vi "FuncVI_Sub - vhShow - Master.vi"() -> ()   [LabVIEW 2021]
doc: "::: CalcExpress Toolkit :::\nCopyright (c) 2000-2026 Konstantin Shifershteyn. All rights reserved."
uses:
  cetypes.llb/VarMan Variable Context Handle.ctl
  <vilib>/Utility/miscctls.llb/LVBoundsTypeDef.ctl
panel:
  out "History":bool
  in  "Reversed":bool=TRUE
  out "Variable":string
  out "h_any":T1(array[cluster]) {"timestamp" format="%<%H:%M:%S%2u\n%d/%m/%Y>T"}
  out "h_a2str":T2(array[cluster]) {"timestamp" format="%<%H:%M:%S%2u\n%d/%m/%Y>T"}
  out "h_a1str":T3(array[cluster]) {"timestamp" format="%<%H:%M:%S%2u\n%d/%m/%Y>T"}
  out "h_a2cdb":T4(array[cluster]) {"value"."data" format="%.2f"; "timestamp" format="%<%H:%M:%S%2u\n%d/%m/%Y>T"}
  out "h_a1cdb":T5(array[cluster]) {"value"."data" format="%.2f"; "timestamp" format="%<%H:%M:%S%2u\n%d/%m/%Y>T"}
  out "h_cdb":T6(array[cluster]) {"value" format="%.2f"; "timestamp" format="%<%H:%M:%S%2u\n%d/%m/%Y>T"}
  out "h_a2dbl":T7(array[cluster]) {"value"."data" format="%.2f"; "timestamp" format="%<%H:%M:%S%2u\n%d/%m/%Y>T"}
  out "h_a1dbl":T8(array[cluster]) {"value"."data" format="%.2f"; "timestamp" format="%<%H:%M:%S%2u\n%d/%m/%Y>T"}
  out "h_dbl":T9(array[cluster]) caption="Variable History" {"value" format="%.2f"; "timestamp" format="%<%H:%M:%S%2u\n%d/%m/%Y>T"}
  out "h_str":T1(array[cluster]) caption="Variable History" {"timestamp" format="%<%H:%M:%S%2u\n%d/%m/%Y>T"}
  in  "name":string
  in  "vch":T10=-1
  in  "update":bool
  in  "Display style":u32(ring) items=["Normal", "'\\' Code", "Password", "Hex dump"]
  in  "Precision":u8=2
  in  "Format":u8(ring) items=["Floating point", "Scientific", "Engineering", "Binary", "Octal", "Hexadecimal", "Relative time", "Absolute time"]
  out "Var Type":i32(ring)=1 items=["String", "DBL Number", "identifier", "1D Array of DBL", "2D Array of DBL", "CDB Number", "1D Array of CDB", "2D Array of CDB", "1D Array of String", "2D Array of String", "Unknown data type"]
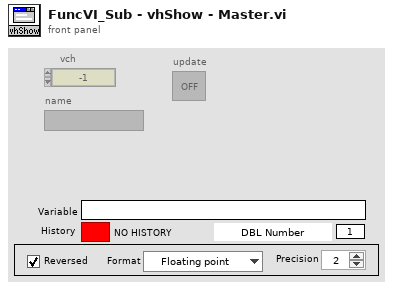
[diagram p1: front panel]
types:
  T1 = cluster{"timestamp":dbl, "value":string, "writerID":u32}[]
  T2 = cluster{"timestamp":dbl, "value":cluster{"data":string[][]}, "writerID":u32}[]
  T3 = cluster{"timestamp":dbl, "value":cluster{"data":string[]}, "writerID":u32}[]
  T4 = cluster{"timestamp":dbl, "value":cluster{"data":cdb[][]}, "writerID":u32}[]
  T5 = cluster{"timestamp":dbl, "value":cluster{"data":cdb[]}, "writerID":u32}[]
  T6 = cluster{"timestamp":dbl, "value":cdb, "writerID":u32}[]
  T7 = cluster{"timestamp":dbl, "value":cluster{"data":dbl[][]}, "writerID":u32}[]
  T8 = cluster{"timestamp":dbl, "value":cluster{"data":dbl[]}, "writerID":u32}[]
  T9 = cluster{"timestamp":dbl, "value":dbl, "writerID":u32}[]
  T10 = typedef "VarMan Variable Context Handle.ctl" = i32
  T11 = typedef "LVBoundsTypeDef.ctl" = cluster{"Width":u32, "Height":u32}
  T12 = typedef "LVPositionTypeDef.ctl" = cluster{"Left":i32, "Top":i32}
  T13 = typedef "eventvkey.ctl" = enum16{"ASCII", "Enter", "Return", "Shift", "Ctrl", "Alt", "Cmd", "Opt", "Caps", "NumLock", "Clear", "Break", "Up", "Down", "Left", "Right", "Insert", "Delete", "Home", "End", "PageUp", "PageDown", "Escape", "Help", "Pause", "ScrollLock", "F1", "F2", "F3", "F4", "F5", "F6", "F7", "F8", "F9", "F10", "F11", "F12", "F13", "F14", "F15", "F16", "F17", "F18", "F19", "F20", "F21", "F22", "F23", "F24", "Play", "VolumeUp", "VolumeDown", "Mute", "Two Byte Char"}
  T14 = cluster{"Shift":bool, "Ctrl":bool, "Alt":bool, "Cmd":bool, "Opt":bool}
  T15 = cluster{"timestamp":dbl, "value":string, "value":u32}[]
  T16 = cluster{"timestamp":dbl, "value":dbl, "value":u32}[]
  T17 = cluster{"timestamp":dbl, "value":cluster{"data":dbl[]}, "value":u32}[]
  T18 = cluster{"timestamp":dbl, "value":cluster{"data":dbl[][]}, "value":u32}[]
  T19 = cluster{"timestamp":dbl, "value":cdb, "value":u32}[]
  T20 = cluster{"timestamp":dbl, "value":cluster{"data":cdb[]}, "value":u32}[]
  T21 = cluster{"timestamp":dbl, "value":cluster{"data":cdb[][]}, "value":u32}[]
  T22 = cluster{"timestamp":dbl, "value":cluster{"data":string[]}, "value":u32}[]
  T23 = cluster{"timestamp":dbl, "value":cluster{"data":string[][]}, "value":u32}[]
  T24 = typedef "LVRectTypeDef.ctl" = cluster{"Left":i16, "Top":i16, "Right":i16, "Bottom":i16}
  T25 = cluster{"Left":i32, "Top":i32, "Right":i32, "Bottom":i32}
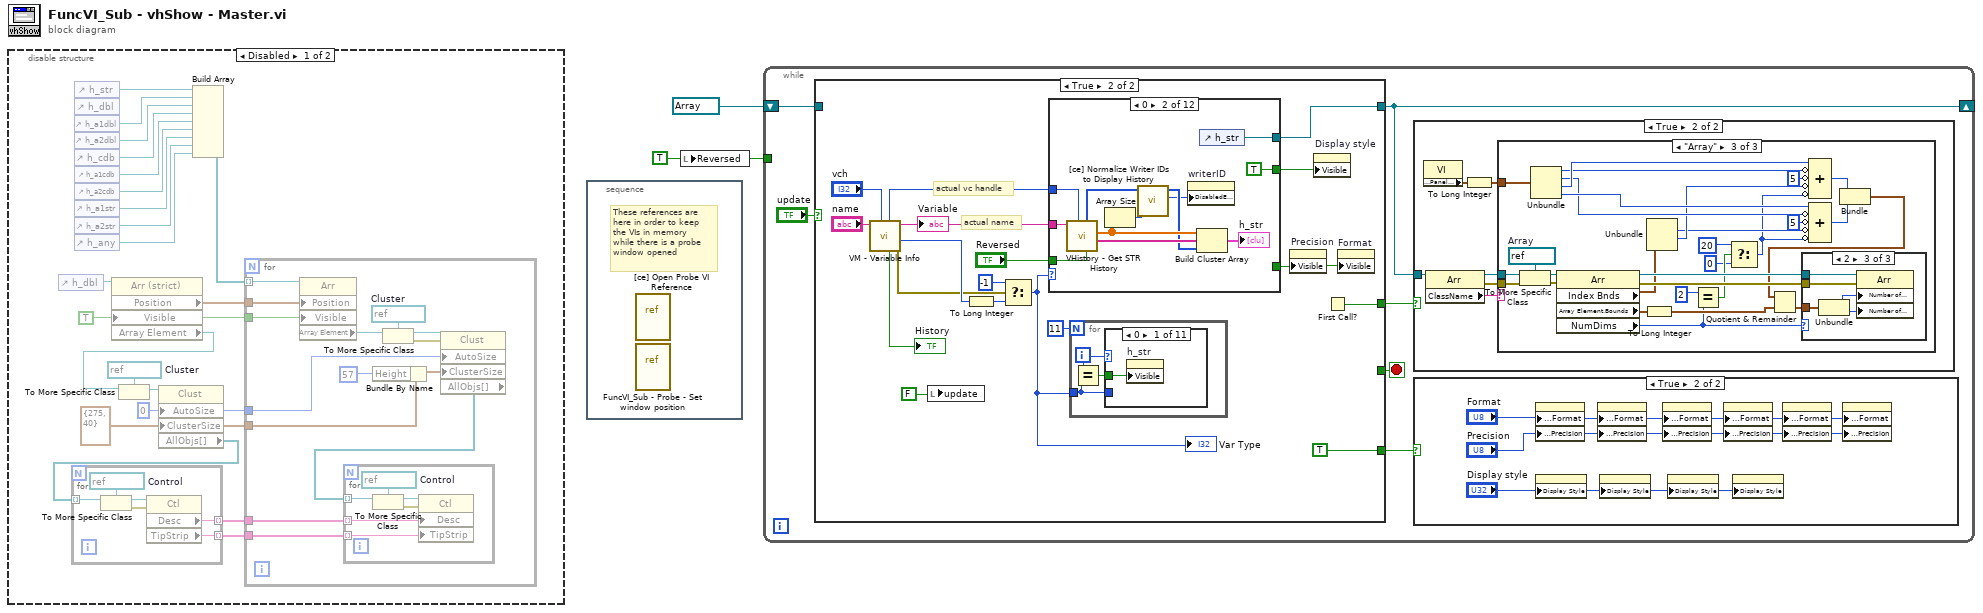
[diagram p0: block diagram]
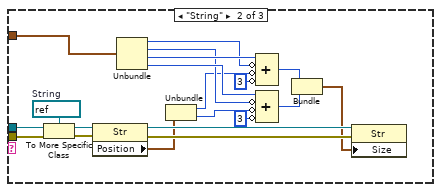
[diagram p5: hidden frame]
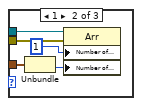
[diagram p7: hidden frame]
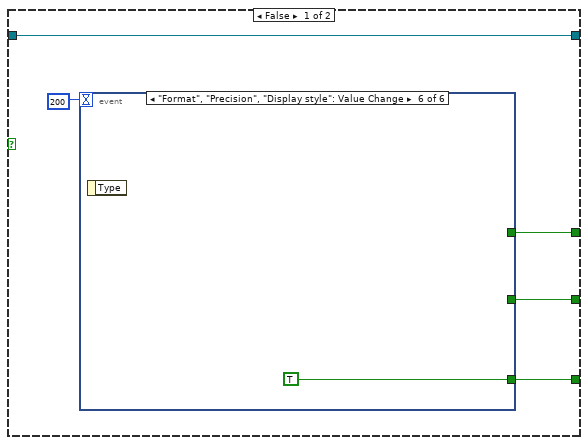
[diagram p9: hidden frame]
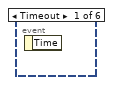
[diagram p10: hidden frame]
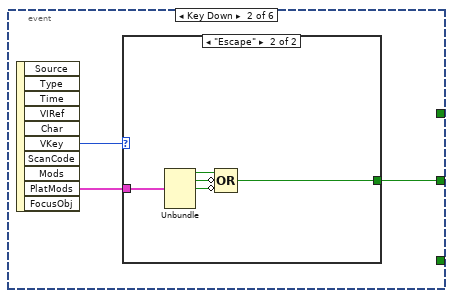
[diagram p11: hidden frame]
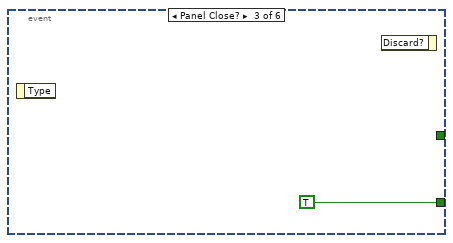
[diagram p13: hidden frame]
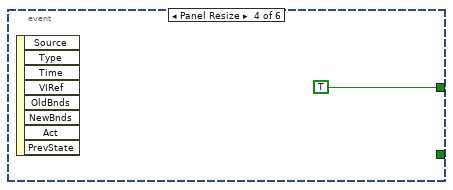
[diagram p14: hidden frame]
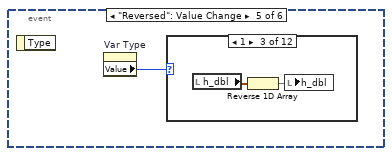
[diagram p15: hidden frame]
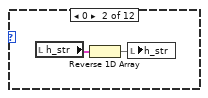
[diagram p17: hidden frame]
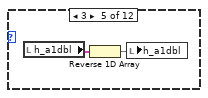
[diagram p19: hidden frame]
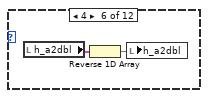
[diagram p20: hidden frame]
diagram:
  w2 = TRUE ("reversed")
  n1 = disable-structure shown="Disabled" {
    frame Disabled {
      w3 = TRUE ("Visible")
      w7 = T11 {"Width"=275, "Height"=40} ("Cluster Size")
      w8 = u32 0 ("Auto Sizing")
      w11 = refnum<vi> refnum  # Cluster
      n2 = control-ref of="h_dbl"() -> (w14:refnum<vi>)
      n3 = control-ref of="h_str"() -> (w23:refnum<vi>)
      n4 = control-ref of="h_dbl"() -> ()  [unwired: 1 out]
      n5 = control-ref of="h_a1dbl"() -> (w22:refnum<vi>)
      n6 = control-ref of="h_a2dbl"() -> (w21:refnum<vi>)
      n7 = control-ref of="h_cdb"() -> (w20:refnum<vi>)
      n8 = control-ref of="h_a1cdb"() -> (w19:refnum<vi>)
      n9 = control-ref of="h_a2cdb"() -> (w18:refnum<vi>)
      n10 = control-ref of="h_a1str"() -> (w17:refnum<vi>)
      n11 = control-ref of="h_a2str"() -> (w16:refnum<vi>)
      n12 = control-ref of="h_any"() -> (w15:refnum<vi>)
      n13 = property class="Arr (strict)"(reference=w14, "Visible"=w3) -> ("Position"=w13:T12, "Array Element"=w10:refnum<vi>)  [unwired: 1 in, 2 out]
      n14 = To More Specific Class(target class=w11, reference=w10) -> (specific class reference=w9:refnum<vi>)  [unwired: 1 in, 1 out]
      n15 = property class="Clust"(reference=w9, "AutoSize"=w8, "ClusterSize"=w7) -> ("AllObjs[]"=w6:refnum<vi>[])  [unwired: 1 in, 2 out]
      n16 = for {
        tunnel: w6 -> [w28] mode=indexing
        tunnel: [w25] -> w5 mode=indexing
        tunnel: [w24] -> w4 mode=indexing
        w29 = refnum<vi> refnum  # Control
        n17 = To More Specific Class(target class=w29, reference=w28) -> (specific class reference=w27:refnum<vi>, error out=w26:errorcluster)  [unwired: 1 in]
        n18 = property class="Ctl"(reference=w27, error in=w26) -> ("Desc"=w25:string, "TipStrip"=w24:string)  [unwired: 2 out]
      }
      n19 = Build Array(w23, w22, w21, w20, w19, w18, w17, w16, w15) -> (w12:refnum<vi>[])
      n20 = for {
        tunnel: w13 -> [w43]
        tunnel: w12 -> [w42] mode=indexing
        tunnel: w8 -> [w37]
        tunnel: w7 -> [w36]
        tunnel: w5 -> [w32]
        tunnel: w4 -> [w31]
        tunnel: w3 -> [w30]
        w41 = refnum<vi> refnum  # Cluster
        n21 = property class="Arr"(reference=w42, "Position"=w43, "Visible"=w30) -> ("Array Element"=w40:refnum<vi>)  [unwired: 1 in, 2 out]
        n22 = Bundle By Name(cluster=w36, "Height"=u32 57) -> (w35:T11)
        n23 = To More Specific Class(target class=w41, reference=w40) -> (specific class reference=w39:refnum<vi>, error out=w38:errorcluster)  [unwired: 1 in]
        n24 = property class="Clust"(reference=w39, error in=w38, "AutoSize"=w37, "ClusterSize"=w35) -> ("AllObjs[]"=w33:refnum<vi>[])  [unwired: 2 out]
        n25 = for {
          tunnel: w33 -> [w48] mode=indexing
          tunnel: w32 -> [w45] mode=indexing
          tunnel: w31 -> [w44] mode=indexing
          w49 = refnum<vi> refnum  # Control
          n26 = To More Specific Class(target class=w49, reference=w48) -> (specific class reference=w47:refnum<vi>, error out=w46:errorcluster)  [unwired: 1 in]
          n27 = property class="Ctl"(reference=w47, error in=w46, "Desc"=w45, "TipStrip"=w44) -> ()  [unwired: 2 out]
        }
      }
    }
    frame Enabled {
    }
  }
  n28 = stacked-sequence {
    frame #0 {
      # "These references are\nhere in order to keep\nthe VIs in memory\nwhile there is a probe\nwindow opened"
      n29 = vi-ref "[ce] Open Probe VI Reference.vi"() -> ()  [unwired: 1 out]
      n30 = vi-ref "FuncVI_Sub - Probe - Set window position.vi"() -> ()  [unwired: 1 out]
    }
  }
  n31 = local write "Reversed"(w2) -> ()
  n32 = while {
    tunnel: w2 -> [_]
    shift-right: [w51] -> _
    shift-left: refnum<vi> refnum ("h_str") -> [w53]
    stop <- w54 stop-if-true
    n33 = case shown="True" "update" {
      tunnel: [w127 _] -> w54
      tunnel: [w126 w162] -> w51
      tunnel: w53 -> [w126 _]
      tunnel: [w125 TRUE] -> w52
      tunnel: [w124 w161] -> w50
      frame False {
        n34 = event shown="[5] \"Format\", \"Precision\", \"Display style\": Value Change" {
          selector: _ -> [_ _ _ _ _ _]
          dyn-events: _ -> [_ _ _ _ _ _]
          timeout: 200 ("millisecond multiple") -> [_ _ _ _ _ _]
          tunnel: [_ w129 TRUE _ _ _] -> w127
          tunnel: [_ _ _ _ _ TRUE] -> w125
          tunnel: [_ _ _ TRUE _ _] -> w124
          event Timeout {
            n35 = event-data() -> ()  [unwired: 1 in, 1 out]
          }
          event Key Down {
            n36 = event-data() -> ("VKey"=w131:T13, "PlatMods"=w130:T14)  [unwired: 1 in, 8 out]
            n37 = case shown="\"Escape\"" w131 {
              tunnel: w130 -> [_ w136]
              tunnel: [_ w132] -> w129
              frame Default {
              }
              frame "Escape" {
                n38 = Unbundle(w136) -> ("Shift"=w135:bool, "Ctrl"=w134:bool, "Alt"=w133:bool)  [unwired: 2 out]
                n39 = Compound Arithmetic op=OR(w135, invert w134, invert w133) -> (w132:bool)
              }
            }
          }
          event Panel Close? {
            n40 = event-data() -> ()  [unwired: 1 in, 1 out]
            n41 = event-data() -> ()  [unwired: 2 in, 1 out]
          }
          event Panel Resize {
            n42 = event-data() -> ()  [unwired: 1 in, 8 out]
          }
          event "Reversed": Value Change {
            n43 = event-data() -> ()  [unwired: 1 in, 1 out]
            n44 = property on="Var Type" class="Ring (strict)"() -> ("Value"=w139:i32)  [unwired: 2 in, 2 out]
            n45 = case shown="1" w139 {
              frame -1 {
              }
              frame 0 {
                n46 = local read "h_str"() -> (w141:T1)
                n47 = Reverse 1D Array(array=w141) -> (reversed array=w140:T1)
                n48 = local write "h_str"(w140) -> ()
              }
              frame 1 {
                n49 = local read "h_dbl"() -> (w143:T9)
                n50 = Reverse 1D Array(array=w143) -> (reversed array=w142:T9)
                n51 = local write "h_dbl"(w142) -> ()
              }
              frame 2 {
              }
              frame 3 {
                n52 = local read "h_a1dbl"() -> (w145:T8)
                n53 = Reverse 1D Array(array=w145) -> (reversed array=w144:T8)
                n54 = local write "h_a1dbl"(w144) -> ()
              }
              frame 4 {
                n55 = local read "h_a2dbl"() -> (w147:T7)
                n56 = Reverse 1D Array(array=w147) -> (reversed array=w146:T7)
                n57 = local write "h_a2dbl"(w146) -> ()
              }
              frame 5 {
                n58 = local read "h_cdb"() -> (w149:T6)
                n59 = Reverse 1D Array(array=w149) -> (reversed array=w148:T6)
                n60 = local write "h_cdb"(w148) -> ()
              }
              frame 6 {
                n61 = local read "h_a1cdb"() -> (w151:T5)
                n62 = Reverse 1D Array(array=w151) -> (reversed array=w150:T5)
                n63 = local write "h_a1cdb"(w150) -> ()
              }
              frame 7 {
                n64 = local read "h_a2cdb"() -> (w153:T4)
                n65 = Reverse 1D Array(array=w153) -> (reversed array=w152:T4)
                n66 = local write "h_a2cdb"(w152) -> ()
              }
              frame 8 {
                n67 = local read "h_a1str"() -> (w155:T3)
                n68 = Reverse 1D Array(array=w155) -> (reversed array=w154:T3)
                n69 = local write "h_a1str"(w154) -> ()
              }
              frame 9 {
                n70 = local read "h_a2str"() -> (w157:T2)
                n71 = Reverse 1D Array(array=w157) -> (reversed array=w156:T2)
                n72 = local write "h_a2str"(w156) -> ()
              }
              frame 10, Default {
                n73 = local read "h_any"() -> (w159:T1)
                n74 = Reverse 1D Array(array=w159) -> (reversed array=w158:T1)
                n75 = local write "h_any"(w158) -> ()
              }
            }
          }
          event "Format", "Precision", "Display style": Value Change {
            n76 = event-data() -> ()  [unwired: 1 in, 1 out]
          }
        }
      }
      frame True {
        # "actual name"
        # "actual vc handle"
        n77 = call "VM - Variable Info.vi"("VC Handle"="vch", "name_spec"="name") -> ("error out"=w163:errorcluster, "var type"=w172:u32, "var name"=w170:string, "has history"=→"History":bool, "var VC Handle"=w167:T10)  [unwired: 4 in, 1 out]
        "Variable" <- w170
        n78 = local write "update"(FALSE ("update")) -> ()
        n79 = To Long Integer(number=w172) -> (32bit integer=w175:i32)
        n80 = Select(t=-1, s=w163, f=w175) -> (s? t:f=w165:i32)
        "Var Type" <- w165
        n81 = case shown="0" w165 {
          tunnel: w170 -> [_ w193 w205 _ w217 w229 w241 w253 w265 w277 w289 w301]
          tunnel: w167 -> [_ w192 w204 _ w216 w228 w240 w252 w264 w276 w288 w300]
          tunnel: "Reversed" -> [_ w189 w200 _ w213 w226 w238 w250 w262 w274 w286 w296]
          tunnel: [_ _ TRUE _ TRUE TRUE TRUE TRUE TRUE _ _ _] -> w173
          tunnel: [_ TRUE _ _ _ _ _ _ _ TRUE TRUE TRUE] -> w171
          tunnel: [_ w187 w199 _ w211 w223 w235 w247 w259 w271 w283 w295] -> w162
          frame -1 {
            n82 = local read "name"() -> (w181:string)
            n83 = Format Into String(format string="ERROR : \"%s\"", w181) -> (resulting string=w179:string)  [unwired: 2 in, 1 out]
            n84 = local write "Variable"(w179) -> ()
          }
          frame 0 {
            n85 = call "VHistory - Get STR History.vi"("reverse order (T)"=w189, "VC Handle"=w192, "name_spec"=w193) -> ("history"=w191:string[], "time stamps"=w185:dbl[], "writer IDs"=w184:u32[])  [unwired: 4 in, 2 out]
            n86 = Array Size(array=w185) -> (size(s)=w186:i32)
            n87 = call "[ce] Normalize Writer IDs to Display History.vi"("size"=w186, "writer IDs in"=w184) -> ("disable"=w182:u8, "writer IDs"=w183:u32[])  [unwired: 8 in]
            n88 = property on="writerID" class="DigNum (strict)"("DisabledEnum"=w182) -> ()  [unwired: 2 in, 2 out]
            n89 = Build Cluster Array(w185, w191, w183) -> (→"h_str":T15)
            n90 = control-ref of="h_str"() -> (w187:refnum<vi>)
          }
          frame 1 {
            n91 = call "VHistory - Get DBL Scalar History.vi"("reverse order (T)"=w200, "VC Handle"=w204, "name_spec"=w205) -> ("history"=w203:dbl[], "time stamps"=w198:dbl[], "writer IDs"=w196:u32[])  [unwired: 4 in, 2 out]
            n92 = Array Size(array=w198) -> (size(s)=w197:i32)
            n93 = call "[ce] Normalize Writer IDs to Display History.vi"("size"=w197, "writer IDs in"=w196) -> ("disable"=w194:u8, "writer IDs"=w195:u32[])  [unwired: 8 in]
            n94 = Build Cluster Array(w198, w203, w195) -> (→"h_dbl":T16)
            n95 = control-ref of="h_dbl"() -> (w199:refnum<vi>)
            n96 = property on="writerID" class="DigNum (strict)"("DisabledEnum"=w194) -> ()  [unwired: 2 in, 2 out]
          }
          frame 2 {
          }
          frame 3 {
            n97 = call "VHistory - Get 1D Array of DBL History.vi"("reverse order (T)"=w213, "VC Handle"=w216, "name_spec"=w217) -> ("history"=w215:cluster{"data":dbl[]}[], "time stamps"=w209:dbl[], "writer IDs"=w208:u32[])  [unwired: 4 in, 2 out]
            n98 = Array Size(array=w209) -> (size(s)=w210:i32)
            n99 = call "[ce] Normalize Writer IDs to Display History.vi"("size"=w210, "writer IDs in"=w208) -> ("disable"=w206:u8, "writer IDs"=w207:u32[])  [unwired: 8 in]
            n100 = Build Cluster Array(w209, w215, w207) -> (→"h_a1dbl":T17)
            n101 = property on="writerID" class="DigNum (strict)"("DisabledEnum"=w206) -> ()  [unwired: 2 in, 2 out]
            n102 = control-ref of="h_a1dbl"() -> (w211:refnum<vi>)
          }
          frame 4 {
            n103 = call "VHistory - Get 2D Array of DBL History.vi"("reverse order (T)"=w226, "VC Handle"=w228, "name_spec"=w229) -> ("history"=w227:cluster{"data":dbl[][]}[], "time stamps"=w221:dbl[], "writer IDs"=w220:u32[])  [unwired: 4 in, 2 out]
            n104 = Array Size(array=w221) -> (size(s)=w222:i32)
            n105 = call "[ce] Normalize Writer IDs to Display History.vi"("size"=w222, "writer IDs in"=w220) -> ("disable"=w218:u8, "writer IDs"=w219:u32[])  [unwired: 8 in]
            n106 = Build Cluster Array(w221, w227, w219) -> (→"h_a2dbl":T18)
            n107 = property on="writerID" class="DigNum (strict)"("DisabledEnum"=w218) -> ()  [unwired: 2 in, 2 out]
            n108 = control-ref of="h_a2dbl"() -> (w223:refnum<vi>)
          }
          frame 5 {
            n109 = call "VHistory - Get CDB Scalar History.vi"("reverse order (T)"=w238, "VC Handle"=w240, "name_spec"=w241) -> ("history"=w239:cdb[], "time stamps"=w233:dbl[], "writer IDs"=w232:u32[])  [unwired: 4 in, 2 out]
            n110 = Array Size(array=w233) -> (size(s)=w234:i32)
            n111 = call "[ce] Normalize Writer IDs to Display History.vi"("size"=w234, "writer IDs in"=w232) -> ("disable"=w230:u8, "writer IDs"=w231:u32[])  [unwired: 8 in]
            n112 = Build Cluster Array(w233, w239, w231) -> (→"h_cdb":T19)
            n113 = property on="writerID" class="DigNum (strict)"("DisabledEnum"=w230) -> ()  [unwired: 2 in, 2 out]
            n114 = control-ref of="h_cdb"() -> (w235:refnum<vi>)
          }
          frame 6 {
            n115 = call "VHistory - Get 1D Array of CDB History.vi"("reverse order (T)"=w250, "VC Handle"=w252, "name_spec"=w253) -> ("history"=w251:cluster{"data":cdb[]}[], "time stamps"=w245:dbl[], "writer IDs"=w244:u32[])  [unwired: 4 in, 2 out]
            n116 = Array Size(array=w245) -> (size(s)=w246:i32)
            n117 = call "[ce] Normalize Writer IDs to Display History.vi"("size"=w246, "writer IDs in"=w244) -> ("disable"=w242:u8, "writer IDs"=w243:u32[])  [unwired: 8 in]
            n118 = Build Cluster Array(w245, w251, w243) -> (→"h_a1cdb":T20)
            n119 = property on="writerID" class="DigNum (strict)"("DisabledEnum"=w242) -> ()  [unwired: 2 in, 2 out]
            n120 = control-ref of="h_a1cdb"() -> (w247:refnum<vi>)
          }
          frame 7 {
            n121 = call "VHistory - Get 2D Array of CDB History.vi"("reverse order (T)"=w262, "VC Handle"=w264, "name_spec"=w265) -> ("history"=w263:cluster{"data":cdb[][]}[], "time stamps"=w257:dbl[], "writer IDs"=w256:u32[])  [unwired: 4 in, 2 out]
            n122 = Array Size(array=w257) -> (size(s)=w258:i32)
            n123 = call "[ce] Normalize Writer IDs to Display History.vi"("size"=w258, "writer IDs in"=w256) -> ("disable"=w254:u8, "writer IDs"=w255:u32[])  [unwired: 8 in]
            n124 = Build Cluster Array(w257, w263, w255) -> (→"h_a2cdb":T21)
            n125 = property on="writerID" class="DigNum (strict)"("DisabledEnum"=w254) -> ()  [unwired: 2 in, 2 out]
            n126 = control-ref of="h_a2cdb"() -> (w259:refnum<vi>)
          }
          frame 8 {
            n127 = call "VHistory - Get 1D Array of STR History.vi"("reverse order (T)"=w274, "VC Handle"=w276, "name_spec"=w277) -> ("history"=w275:cluster{"data":string[]}[], "time stamps"=w269:dbl[], "writer IDs"=w268:u32[])  [unwired: 4 in, 2 out]
            n128 = Array Size(array=w269) -> (size(s)=w270:i32)
            n129 = call "[ce] Normalize Writer IDs to Display History.vi"("size"=w270, "writer IDs in"=w268) -> ("disable"=w266:u8, "writer IDs"=w267:u32[])  [unwired: 8 in]
            n130 = property on="writerID" class="DigNum (strict)"("DisabledEnum"=w266) -> ()  [unwired: 2 in, 2 out]
            n131 = Build Cluster Array(w269, w275, w267) -> (→"h_a1str":T22)
            n132 = control-ref of="h_a1str"() -> (w271:refnum<vi>)
          }
          frame 9 {
            n133 = call "VHistory - Get 2D Array of STR History.vi"("reverse order (T)"=w286, "VC Handle"=w288, "name_spec"=w289) -> ("history"=w287:cluster{"data":string[][]}[], "time stamps"=w281:dbl[], "writer IDs"=w280:u32[])  [unwired: 4 in, 2 out]
            n134 = Array Size(array=w281) -> (size(s)=w282:i32)
            n135 = call "[ce] Normalize Writer IDs to Display History.vi"("size"=w282, "writer IDs in"=w280) -> ("disable"=w278:u8, "writer IDs"=w279:u32[])  [unwired: 8 in]
            n136 = property on="writerID" class="DigNum (strict)"("DisabledEnum"=w278) -> ()  [unwired: 2 in, 2 out]
            n137 = Build Cluster Array(w281, w287, w279) -> (→"h_a2str":T23)
            n138 = control-ref of="h_a2str"() -> (w283:refnum<vi>)
          }
          frame 10, Default {
            n139 = call "VHistory - Get Arbitrary Variable History.vi"("reverse order (T)"=w296, "VC Handle"=w300, "name_spec"=w301) -> ("history"=w299:string[], "time stamps"=w293:dbl[], "writer IDs"=w292:u32[])  [unwired: 4 in, 2 out]
            n140 = Array Size(array=w293) -> (size(s)=w294:i32)
            n141 = call "[ce] Normalize Writer IDs to Display History.vi"("size"=w294, "writer IDs in"=w292) -> ("disable"=w290:u8, "writer IDs"=w291:u32[])  [unwired: 8 in]
            n142 = property on="writerID" class="DigNum (strict)"("DisabledEnum"=w290) -> ()  [unwired: 2 in, 2 out]
            n143 = Build Cluster Array(w293, w299, w291) -> (→"h_any":T15)
            n144 = control-ref of="h_any"() -> (w295:refnum<vi>)
          }
        }
        n145 = for {
          N: 11 -> [_]
          tunnel: w165 -> [w302]
          i -> [w303]
          n146 = Equal?(x=w303, y=w302) -> (x = y?=w304:bool)
          n147 = case shown="0" w303 {
            selector: w303 -> [_ _ _ _ _ _ _ _ _ _ w316]
            tunnel: w304 -> [w305 w306 _ w307 w308 w309 w310 w311 w312 w313 _]
            tunnel: w302 -> [_ _ _ _ _ _ _ _ _ _ w315]
            frame 0 {
              n148 = property on="h_str" class="Arr (strict)"("Visible"=w305) -> ()  [unwired: 2 in, 2 out]
            }
            frame 1 {
              n149 = property on="h_dbl" class="Arr (strict)"("Visible"=w306) -> ()  [unwired: 2 in, 2 out]
            }
            frame 2 {
            }
            frame 3 {
              n150 = property on="h_a1dbl" class="Arr (strict)"("Visible"=w307) -> ()  [unwired: 2 in, 2 out]
            }
            frame 4 {
              n151 = property on="h_a2dbl" class="Arr (strict)"("Visible"=w308) -> ()  [unwired: 2 in, 2 out]
            }
            frame 5 {
              n152 = property on="h_cdb" class="Arr (strict)"("Visible"=w309) -> ()  [unwired: 2 in, 2 out]
            }
            frame 6 {
              n153 = property on="h_a1cdb" class="Arr (strict)"("Visible"=w310) -> ()  [unwired: 2 in, 2 out]
            }
            frame 7 {
              n154 = property on="h_a2cdb" class="Arr (strict)"("Visible"=w311) -> ()  [unwired: 2 in, 2 out]
            }
            frame 8 {
              n155 = property on="h_a1str" class="Arr (strict)"("Visible"=w312) -> ()  [unwired: 2 in, 2 out]
            }
            frame 9 {
              n156 = property on="h_a2str" class="Arr (strict)"("Visible"=w313) -> ()  [unwired: 2 in, 2 out]
            }
            frame 10, Default {
              n157 = Less Or Equal?(x=w316, y=w315) -> (x <= y?=w314:bool)
              n158 = property on="h_any" class="Arr (strict)"("Visible"=w314) -> ()  [unwired: 2 in, 2 out]
            }
          }
        }
        n159 = property on="Precision" class="DigNum (strict)"("Visible"=w173) -> ()  [unwired: 2 in, 2 out]
        n160 = property on="Display style" class="Ring (strict)"("Visible"=w171) -> ()  [unwired: 2 in, 2 out]
        n161 = First Call?() -> (First Call?: T/F=w161:bool)
        n162 = property on="Format" class="Ring (strict)"("Visible"=w173) -> ()  [unwired: 2 in, 2 out]
      }
    }
    n163 = case shown="True" w50 {
      tunnel: w51 -> [_ w61]
      frame False {
      }
      frame True {
        n164 = property on="Property Node" class="VI"() -> ("Front Panel.PanelBounds"=w57:T24)  [unwired: 2 in, 2 out]
        n165 = property on="Property Node" class="Arr"(reference=w61) -> (reference out=w59:refnum<vi>, error out=w58:errorcluster, "ClassName"=w60:string)  [unwired: 1 in]
        n166 = To Long Integer(number=w57) -> (32bit integer=w56:T25)
        n167 = case shown="\"Array\"" w60 {
          tunnel: w59 -> [_ w81 w110]
          tunnel: w58 -> [_ w66 w101]
          tunnel: w56 -> [_ w63 w98]
          frame Default {
          }
          frame "String" {
            w80 = refnum<vi> refnum  # String
            n168 = To More Specific Class(target class=w80, reference=w81, error in=w66) -> (specific class reference=w65:refnum<vi>, error out=w64:errorcluster)
            n169 = property on="Property Node" class="Str"(reference=w65, error in=w64) -> (reference out=w78:refnum<vi>, error out=w79:errorcluster, "Position"=w77:T12)
            n170 = Unbundle(w63) -> ("Left"=w62:i32, "Top"=w74:i32, "Right"=w76:i32, "Bottom"=w75:i32)
            n171 = Unbundle(w77) -> ("Left"=w73:i32, "Top"=w72:i32)
            n172 = Compound Arithmetic op=ADD(w76, invert w62, invert w73, invert 3 ("value")) -> (w71:i32)
            n173 = Compound Arithmetic op=ADD(w75, invert w74, invert w72, invert 3 ("value")) -> (w70:i32)
            n174 = Bundle(w71, w70) -> (w69:cluster{i32, i32})  [unwired: 1 in]
            n175 = property on="Property Node" class="Str"(reference=w78, error in=w79, "Size"=w69) -> ()  [unwired: 2 out]
          }
          frame "Array" {
            w109 = refnum<vi> refnum  # Array
            n176 = To More Specific Class(target class=w109, reference=w110, error in=w101) -> (specific class reference=w100:refnum<vi>, error out=w99:errorcluster)
            n177 = Unbundle(w98) -> ("Left"=w97:i32, "Top"=w104:i32, "Right"=w106:i32, "Bottom"=w105:i32)
            n178 = property on="Property Node" class="Arr"(reference=w100, error in=w99) -> (reference out=w107:refnum<vi>, error out=w108:errorcluster, "Index Bnds"=w91:T24, "Array Element.Bounds"=w96:T11, "NumDims"=w83:u32)
            n179 = To Long Integer(number=w96) -> (32bit integer=w93:cluster{"Width":i32, "Height":i32})
            n180 = Unbundle(w91) -> ("Top"=w89:i16, "Right"=w90:i16)  [unwired: 2 out]
            n181 = Equal?(x=u32 2 ("y"), y=w83) -> (x = y?=w87:bool)
            n182 = Select(t=20 ("value"), s=w87, f=0) -> (s? t:f=w82:i32)
            n183 = Compound Arithmetic op=ADD(w106, invert w97, invert 5 ("value"), invert w90, invert w82) -> (w103:i32)
            n184 = Compound Arithmetic op=ADD(w105, invert w104, invert 5 ("value"), invert w89, invert w82) -> (w102:i32)
            n185 = Bundle(w103, w102) -> (w88:cluster{i32, i32})  [unwired: 1 in]
            n186 = Quotient & Remainder(x=w88, y=w93) -> (floor(x/y)=w92:cluster{i32, i32})  [unwired: 1 out]
            n187 = case shown="2" w83 {
              tunnel: w108 -> [_ w115 w120]
              tunnel: w107 -> [_ w114 w119]
              tunnel: w92 -> [_ w113 w118]
              frame 0, Default {
              }
              frame 1 {
                n188 = Unbundle(w113) -> (w112:i32)  [unwired: 1 out]
                n189 = property on="Property Node" class="Arr"(reference=w114, error in=w115, "Number of Columns"=u32 1, "Number of Rows"=w112) -> ()  [unwired: 2 out]
              }
              frame 2 {
                n190 = Unbundle(w118) -> (w117:i32, w116:i32)
                n191 = property on="Property Node" class="Arr"(reference=w119, error in=w120, "Number of Columns"=w117, "Number of Rows"=w116) -> ()  [unwired: 2 out]
              }
            }
          }
        }
      }
    }
    n192 = case shown="True" w52 {
      frame False {
      }
      frame True {
        n193 = property on="value" class="DigNum (strict)"("Display Format:Format"="Format", "Display Format:Precision"="Precision") -> ()  [unwired: 2 in, 2 out]
        n194 = property on="value" class="Str"("Display Style"="Display style") -> ()  [unwired: 2 in, 2 out]
        n195 = property class="DigNum (strict)"("Display Format:Format"="Format", "Display Format:Precision"="Precision") -> ()  [unwired: 2 in, 2 out]
        n196 = property class="Str"("Display Style"="Display style") -> ()  [unwired: 2 in, 2 out]
        n197 = property on="value" class="DigNum (strict)"("Display Format:Format"="Format", "Display Format:Precision"="Precision") -> ()  [unwired: 2 in, 2 out]
        n198 = property class="Str"("Display Style"="Display style") -> ()  [unwired: 2 in, 2 out]
        n199 = property class="DigNum (strict)"("Display Format:Format"="Format", "Display Format:Precision"="Precision") -> ()  [unwired: 2 in, 2 out]
        n200 = property on="value" class="Str"("Display Style"="Display style") -> ()  [unwired: 2 in, 2 out]
        n201 = property class="DigNum (strict)"("Display Format:Format"="Format", "Display Format:Precision"="Precision") -> ()  [unwired: 2 in, 2 out]
        n202 = property class="DigNum (strict)"("Display Format:Format"="Format", "Display Format:Precision"="Precision") -> ()  [unwired: 2 in, 2 out]
      }
    }
  }
